vi "optical_1.vi"() -> ()   [LabVIEW 2025]
panel:
  out "Optical saving error":errorcluster
  out "Optical Loop Speed (ms)":u32
  in  "STOP ACQUISITION":bool
  out "Optical Frame Out":string
  out "Optical Preview":T1(plugin-control)
  in  "Output Folder":path
  # "^ append to base data folder \"...\\raw\\test_n\" for nth recording"
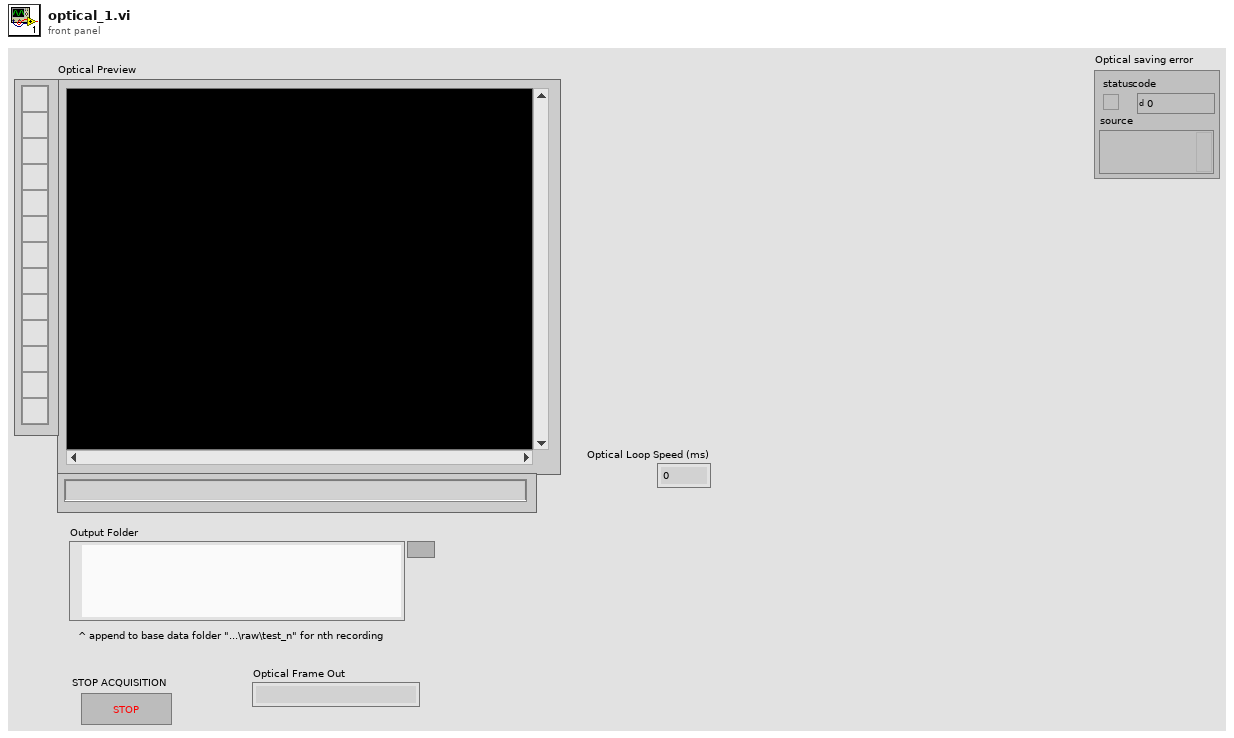
[diagram p1: front panel]
types:
  T1 = typedef "IMAQ Image.ctl" = refnum<image>
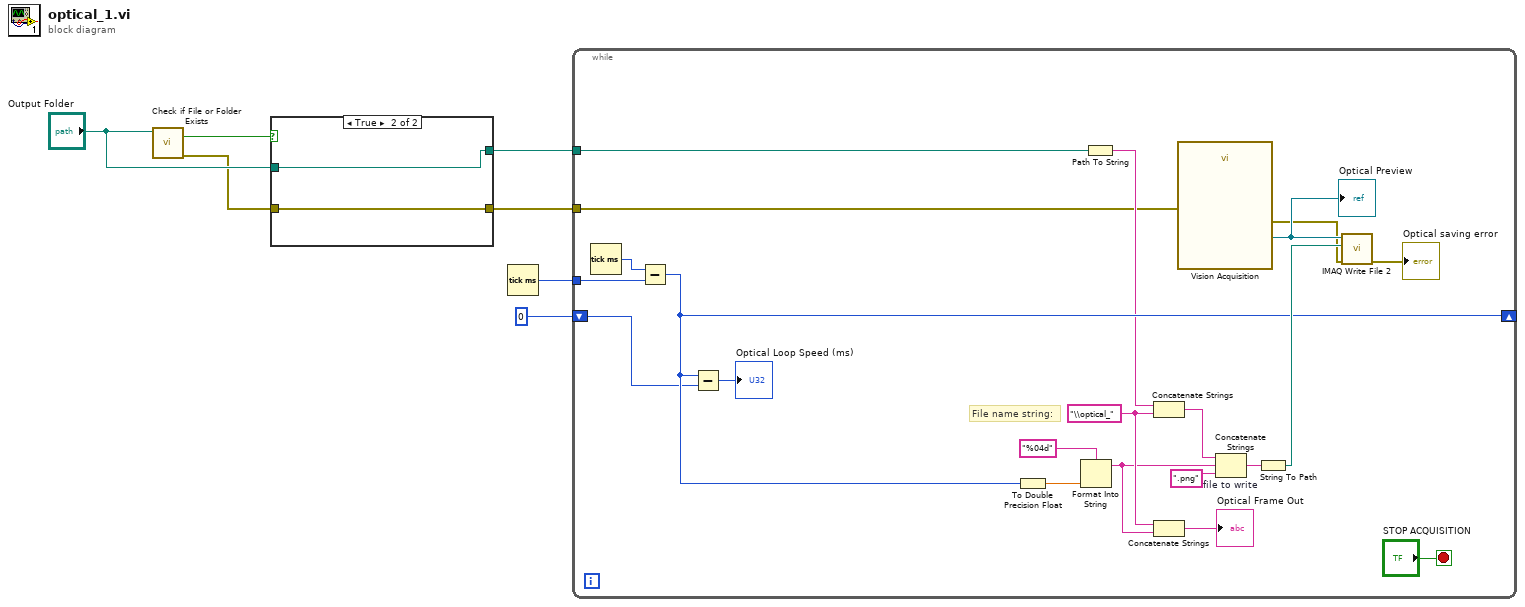
[diagram p0: block diagram]
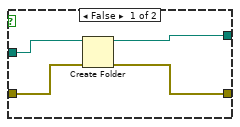
[diagram p2: hidden frame]
diagram:
  n1 = call <vilib>:"Check if File or Folder Exists.vi"("path"="Output Folder") -> ("error out"=w2:errorcluster, "file or folder exists?"=w5:bool)  [unwired: 8 in, 1 out]
  n2 = case shown="True" w5 {
    tunnel: "Output Folder" -> [w11 w13]
    tunnel: [w10 w13] -> w3
    tunnel: w2 -> [w9 w12]
    tunnel: [w8 w12] -> w1
    frame False {
      n3 = Create Folder(path (use dialog)=w11, error in=w9) -> (created path=w10:path, error out=w8:errorcluster)  [unwired: 1 in, 1 out]
    }
    frame True {
    }
  }
  n4 = Tick Count (ms)() -> (millisecond timer value=w7:u32)
  n5 = while {
    tunnel: w7 -> [w22]
    shift-right: [w21] -> _
    shift-left: u32 0 -> [w20]
    tunnel: w3 -> [w16]
    tunnel: w1 -> [w17]
    stop <- "STOP ACQUISITION" stop-if-true
    w30 = "\\optical_" ("string")
    # "File name string:"
    n6 = Tick Count (ms)() -> (millisecond timer value=w23:u32)
    n7 = Subtract(x=w23, y=w22) -> (x-y=w21:u32)
    n8 = Subtract(x=w21, y=w20) -> (x-y=→"Optical Loop Speed (ms)":u32)
    n9 = To Double Precision Float(number=w21) -> (double precision float=w28:dbl)
    n10 = Format Into String(format string="%04d" ("time format string (%c)"), w28) -> (resulting string=w26:string)  [unwired: 2 in, 1 out]
    n11 = Path To String(path=w16) -> (string=w18:string)
    n12 = Concatenate Strings(w18, w30) -> (w31:string)
    n13 = Concatenate Strings(w30, w26) -> (→"Optical Frame Out":string)
    n14 = call "Vision Acquisition"("error in"=w17) -> ("Image Out"=w34:T1, "error out"=w15:errorcluster)  [unwired: 25 in]
    "Optical Preview" <- w34
    n15 = Concatenate Strings "file to write"(w31, w26, ".png" ("string")) -> (w33:string)
    n16 = String To Path(string=w33) -> (path=w27:path)
    n17 = call-poly "IMAQ Write File 2"("error in (no error)"=w15, "File Path"=w27, "Image"=w34) -> ("error out"=→"Optical saving error":errorcluster)  [unwired: 7 in, 1 out]
  }
